vi "Load Section and Instruction.vi"(10 "TestCaseIndex":i32, 11 "TestProcedureMetadata":T1) -> (2 "Instruction":string, 3 "Section":string)   [LabVIEW 2026, in "testCoordinator.lvlib"]
uses:
  testCoordinator.lvlib
  Test Procedure.ctl
panel:
  out "number":u32
  out "cleanup group":bool
  out "main group":bool
  out "setup group":bool
  out "result":i32
  out "TestProcedureMetadata 2":T1
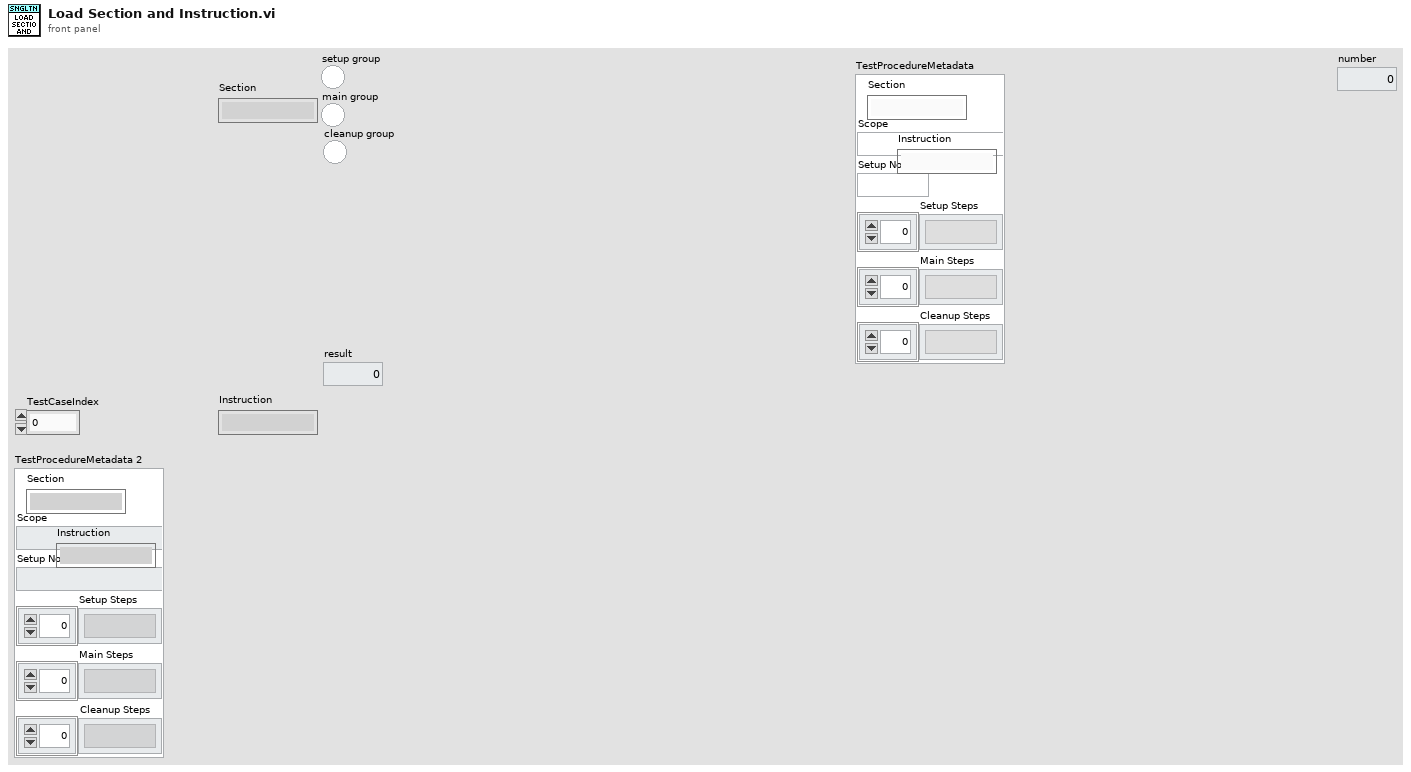
[diagram p1: front panel]
types:
  T1 = typedef "Test Procedure.ctl" = cluster{"Scope":string, "Setup Note":string, "Setup Steps":string[], "Main Steps":string[], "Cleanup Steps":string[], "Section":string, "Instruction":string}
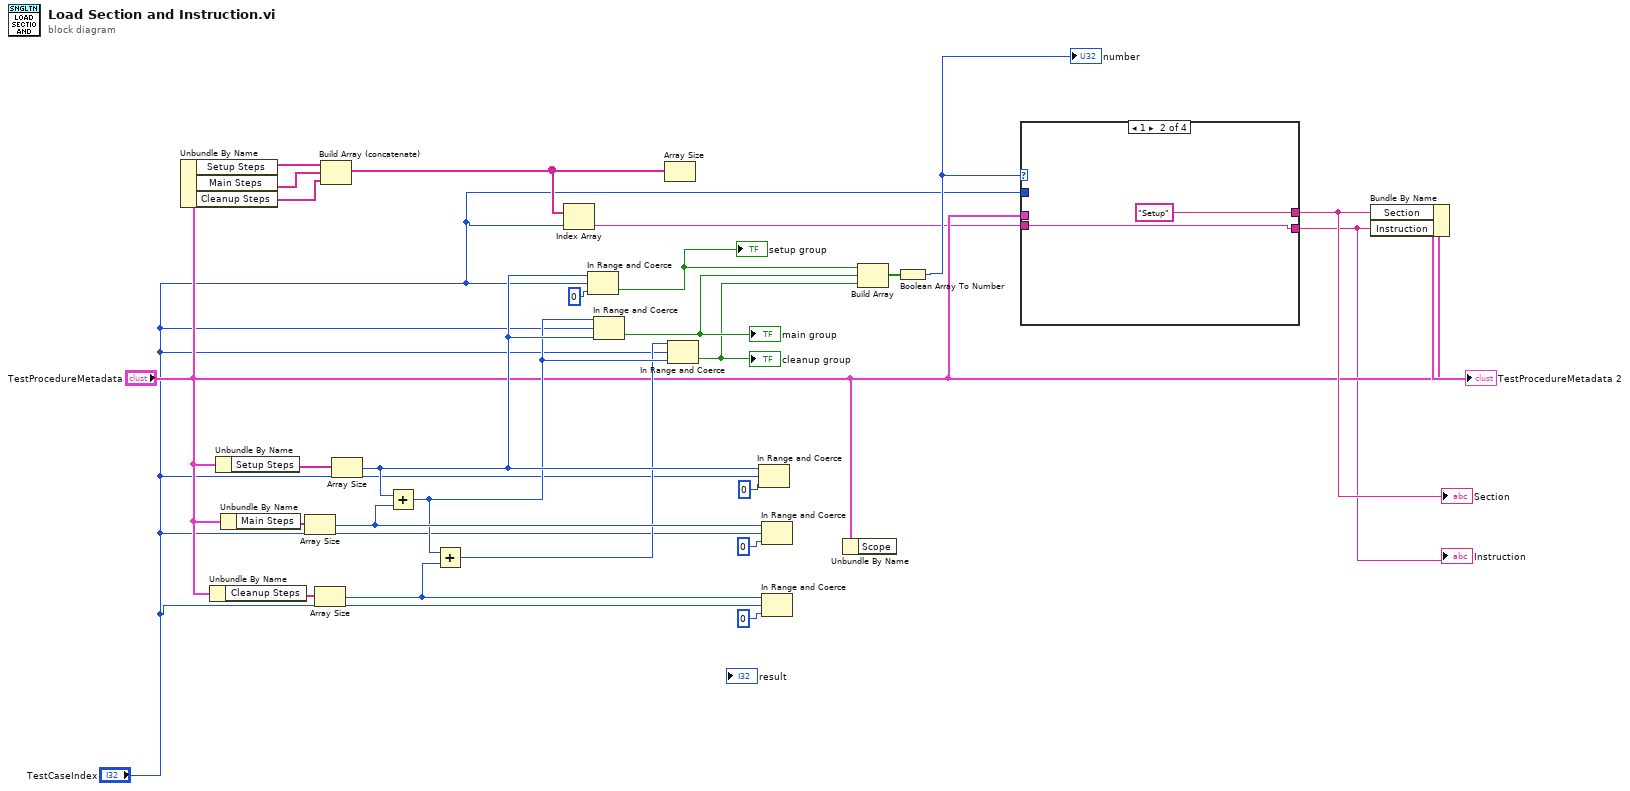
[diagram p0: block diagram]
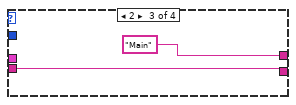
[diagram p3: hidden frame]
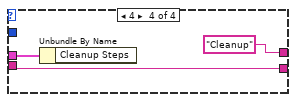
[diagram p4: hidden frame]
diagram:
  n1 = Unbundle By Name("TestProcedureMetadata") -> ("Setup Steps"=w21:string[], "Main Steps"=w20:string[], "Cleanup Steps"=w19:string[])
  n2 = Unbundle By Name("TestProcedureMetadata") -> ("Cleanup Steps"=w22:string[])
  n3 = Unbundle By Name("TestProcedureMetadata") -> ("Setup Steps"=w26:string[])
  n4 = Unbundle By Name("TestProcedureMetadata") -> ("Main Steps"=w25:string[])
  n5 = Array Size(array=w25) -> (size(s)=w18:i32)
  n6 = Array Size(array=w22) -> (size(s)=w17:i32)
  n7 = Build Array (concatenate)(w21, w20, w19) -> (w4:string[])
  n8 = Array Size(array=w26) -> (size(s)=w15:i32)
  n9 = Add(x=w15, y=w18) -> (x+y=w14:i32)
  n10 = Add(x=w14, y=w17) -> (x+y=w13:i32)
  n11 = Index Array(array=w4, index="TestCaseIndex") -> (element=w2:string)
  n12 = In Range and Coerce(upper limit=w15, x="TestCaseIndex", lower limit=0 ("size(s)")) -> (In Range?=w11:bool)  [unwired: 1 out]
  "setup group" <- w11
  n13 = In Range and Coerce(upper limit=w14, x="TestCaseIndex", lower limit=w15) -> (In Range?=w10:bool)  [unwired: 1 out]
  "main group" <- w10
  n14 = Array Size(array=w4) -> ()  [unwired: 1 out]
  n15 = In Range and Coerce(upper limit=w13, x="TestCaseIndex", lower limit=w14) -> (In Range?=w9:bool)  [unwired: 1 out]
  "cleanup group" <- w9
  n16 = In Range and Coerce(upper limit=w15, x="TestCaseIndex", lower limit=0 ("size(s)")) -> ()  [unwired: 2 out]
  n17 = In Range and Coerce(upper limit=w18, x="TestCaseIndex", lower limit=0 ("size(s)")) -> ()  [unwired: 2 out]
  n18 = In Range and Coerce(upper limit=w17, x="TestCaseIndex", lower limit=0 ("size(s)")) -> ()  [unwired: 2 out]
  n19 = Unbundle By Name("TestProcedureMetadata") -> ()  [unwired: 1 out]
  n20 = Build Array(w11, w10, w9) -> (w8:bool[])
  n21 = Boolean Array To Number(Boolean array=w8) -> (number=w7:u32)
  "number" <- w7
  n22 = case shown="1" w7 {
    tunnel: [_ "Setup" ("Section") "Main" ("Section") "Cleanup" ("Section")] -> w6
    tunnel: "TestProcedureMetadata" -> [_ _ _ w34]
    tunnel: "TestCaseIndex" -> [_ _ _ _]
    tunnel: w2 -> [w28 w29 w31 w33]
    tunnel: [w28 w29 w31 w33] -> w1
    frame Default {
    }
    frame 1 {
    }
    frame 2 {
    }
    frame 4 {
      n23 = Unbundle By Name(w34) -> ()  [unwired: 1 out]
    }
  }
  "Section" <- w6
  "Instruction" <- w1
  n24 = Bundle By Name(cluster="TestProcedureMetadata", "Section"=w6, "Instruction"=w1) -> (→"TestProcedureMetadata 2":T1)
